vi "Test Overrides Has Case Structure Removed.vi"(8 "error in (no error)":errorcluster, 11 "Test Case In":refnum<class "_Mock Class Generator Test.lvclass">) -> (0 "error out":errorcluster, 3 "Test Case Out":refnum<class "_Mock Class Generator Test.lvclass">)   [LabVIEW 2020, in "_Mock Class Generator Test.lvclass"]
uses:
  _Mock Class Generator Test.lvclass
  C:/Program Files (x86)/National Instruments/LabVIEW 2020/vi.lib/Astemes/LUnit/Test Case.lvclass
  <vilib>/Utility/traverseref.llb/TRef TravTarget.ctl
  <vilib>/Astemes/LUnit/Test Case.lvclass/Test Case.ctl
  <vilib>/Astemes/LUnit/Append Fail Result.vi
  <vilib>/Astemes/LUnit/Append Pass Result.vi
  <vilib>/Astemes/LUnit/Run In UI.vi
  <vilib>/Utility/error.llb/Clear Errors.vi
  _Mock Class Generator Test.lvclass/_Mock Class Generator Test.ctl
  source/Scripting/Mock Class Generator/Mock Class Generator.lvclass
  <vilib>/Utility/traverseref.llb/VI Scripting - Traverse.lvlib
  <vilib>/Astemes/LUnit/Test Case.lvclass
  C:/Program Files (x86)/National Instruments/LabVIEW 2020/vi.lib/Astemes/LUnit/LUnit Runnable.lvclass
  C:/git/astemes-lmock/tests/Mock Class Generator Test/_Mock Class Generator Test.lvclass
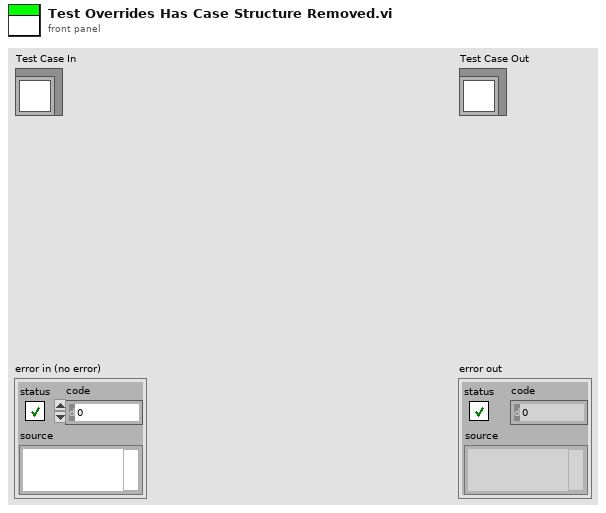
[diagram p1: front panel]
types:
  T1 = typedef "TRef TravTarget.ctl" = enum16{"FP", "BD", "Other"}
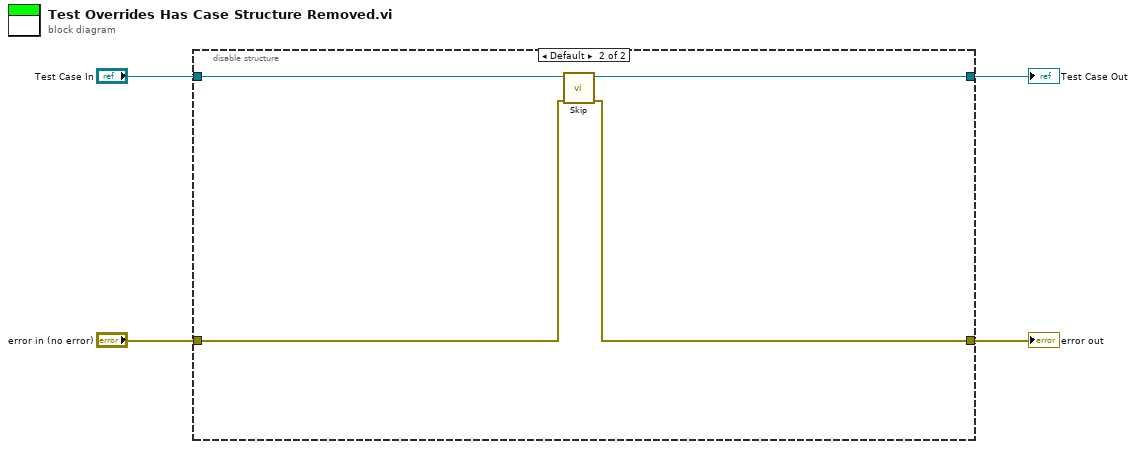
[diagram p0: block diagram]
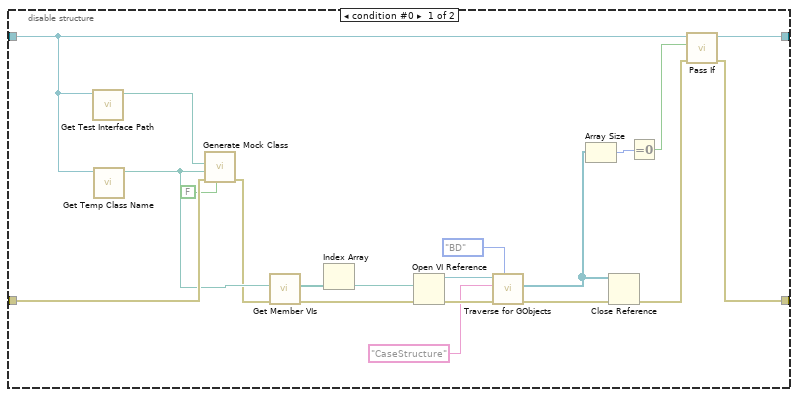
[diagram p2: hidden frame]
diagram:
  n1 = disable-structure shown="Default" {
    disable-tunnel: [w24 w26] -> w4
    disable-tunnel: [w23 w25] -> w3
    disable-tunnel: "Test Case In" -> [w22 w28]
    disable-tunnel: "error in (no error)" -> [w21 w27]
    frame condition #0 {
      n2 = call "Get Test Interface Path.vi"("Mock Class Generator Test in"=w22) -> ("Test Class Path"=w20:path)  [unwired: 10 in]
      n3 = call "Get Temp Class Name.vi"("Mock Class Generator Test in"=w22) -> ("Test Class Path"=w19:path)  [unwired: 10 in]
      n4 = call "Generate Mock Class.vi"("Add to lvproj?"=FALSE, "error in (no error)"=w21, "Destination Class Path"=w19, "Source Class Path"=w20) -> ("error out"=w18:errorcluster)  [unwired: 6 in, 1 out]
      n5 = call "Get Member VIs.vi"("error in (no error)"=w18, "Test Class Path"=w19) -> ("error out"=w17:errorcluster, "Array"=w16:path[])  [unwired: 8 in]
      n6 = Index Array(array=w16) -> (element=w14:path)  [unwired: 1 in]
      n7 = Open VI Reference(vi path=w14, error in (no error)=w17) -> (vi reference=w13:refnum<vi>, error out=w15:errorcluster)  [unwired: 4 in]
      n8 = call <vilib>:"Traverse for GObjects.vi"("Traverse Target"=TRef_TravTarget."BD", "error in (no error)"=w15, "Class Name"="CaseStructure", "VI Refnum"=w13) -> ("error out"=w10:errorcluster, "References"=w6:refnum<vi>[])  [unwired: 4 in, 2 out]
      n9 = Array Size(array=w6) -> (size(s)=w9:i32)
      n10 = Close Reference(reference=w6, error in (no error)=w10) -> (error out=w7:errorcluster)
      n11 = Equal To 0?(x=w9) -> (x = 0?=w8:bool)
      n12 = call <vilib>:"Pass If.vi"("error in (no error)"=w7, "Pass?"=w8, "LUnit Test Case In"=w22) -> ("error out"=w23:errorcluster, "LUnit Test Case Out"=w24:refnum<class "_Mock Class Generator Test.lvclass">)  [unwired: 7 in]
    }
    frame condition #1 (active) {
      n13 = call <vilib>:"Skip.vi"("error in (no error)"=w27, "LUnit Test Case In"=w28) -> ("error out"=w25:errorcluster, "LUnit Test Case Out"=w26:refnum<class "_Mock Class Generator Test.lvclass">)  [unwired: 8 in]
    }
  }
  "error out" <- w3
  "Test Case Out" <- w4
